vi "Path as Path (LabVIEW Path).vi"(10 "Path":path) -> (2 "Path":path)   [LabVIEW 2020, in "G-Unicode.lvlib"]
doc: "Converts the input path to a raw UTF-8 encoded LabVIEW path. Valid inputs are a UTF-8 Path class or LabVIEW path."
uses:
  G-Unicode.lvlib
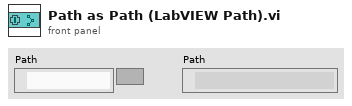
[diagram p1: front panel]
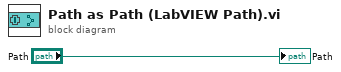
[diagram p0: block diagram]
diagram:
  "Path" <- "Path"
